vi "Register for gRPC Server Events.vi"(8 "error in (no error)":errorcluster, 11 "CIFPlugin in":refnum<class "CAN_Reader_CANsub_Plugin.lvclass">) -> (0 "error out":errorcluster, 2 "Event Registration Refnum":refnum<event-registration>, 3 "CIFPlugin out":refnum<class "CAN_Reader_CANsub_Plugin.lvclass">)   [LabVIEW 2021, in "CAN_Reader_CANsub_Plugin.lvclass"]
uses:
  CAN_Reader_CANsub_Plugin.lvclass
  CAN_Reader_CANsub_Plugin.lvclass/CAN_Reader_CANsub_Plugin.ctl
  <vilib>/CIF Foundation/CIF Core/CIFCore/Class/CIFCorePlugin.lvclass
  Grpc/CanReaderCansub_server/RPC Service/CanReaderCansub/CanReaderCansub.lvclass
  C:/Program Files/National Instruments/LabVIEW 2021/vi.lib/CIF Foundation/CIF Core/CIFCore/Class/CIFCorePlugin.lvclass
  D:/dev/Plugins/CAN_Reader_CANsub/Class/CAN_Reader_CANsub_Plugin.lvclass
  <vilib>/CIF Foundation/CIF U8 Array Monitor gRPC/U8_Array_Monitor_gRPC/CIFU8ArrayMonitorUtilities/CIFU8ArrayMonitorUtilities.lvlib
  C:/Program Files/National Instruments/LabVIEW 2021/vi.lib/gRPC/LabVIEW gRPC Servicer/ServiceBase/ServiceBase.lvclass
  D:/dev/Plugins/CAN_Reader_CANsub/Grpc/CanReaderCansub_server/RPC Service/CanReaderCansub/CanReaderCansub.lvclass
  <vilib>/gRPC/LabVIEW gRPC Library/Shared/grpcId.ctl
  <vilib>/gRPC/LabVIEW gRPC Library/grpc-lvsupport-release.lvlib
  <vilib>/gRPC/LabVIEW gRPC Library/Server API/typeDefs/gRPCId Cluster.ctl
  <vilib>/CIF Foundation/CIF U8 Array Monitor gRPC/U8_Array_Monitor_gRPC/CIFU8ArrayMonitor_server/RPC Service/U8ArrayMonitor/typeDefs/Server gRPC UEs.ctl
  <vilib>/CIF Foundation/CIF U8 Array Monitor gRPC/U8_Array_Monitor_gRPC/CIFU8ArrayMonitor_server/RPC Service/U8ArrayMonitor/U8ArrayMonitor.lvclass
  Grpc/CanReaderCansub_server/RPC Service/CanReaderCansub/typeDefs/Server gRPC UEs.ctl
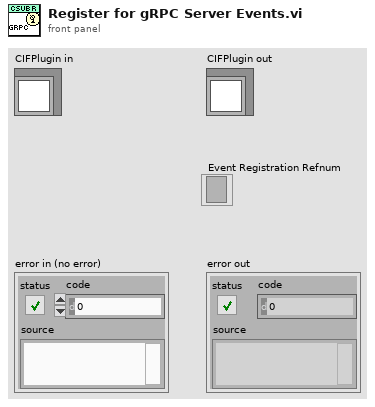
[diagram p1: front panel]
types:
  T1 = typedef "CIFU8ArrayMonitor_server.lvlib/U8ArrayMonitor.lvclass/Server gRPC UEs.ctl" = cluster{"U8ArrayMonitor SetEnableU8Array gRPC UE":refnum<user-event>, "U8ArrayMonitor GetU8Array gRPC UE":refnum<user-event>}
  T2 = typedef "CanReaderCansub_server.lvlib/CanReaderCansub.lvclass/Server gRPC UEs.ctl" = cluster{"CanReaderCansub GetDevices gRPC UE":refnum<user-event>, "CanReaderCansub GetStatistics gRPC UE":refnum<user-event>, "CanReaderCansub SetInterfaceBlink gRPC UE":refnum<user-event>, "CanReaderCansub GetCANStatus gRPC UE":refnum<user-event>}
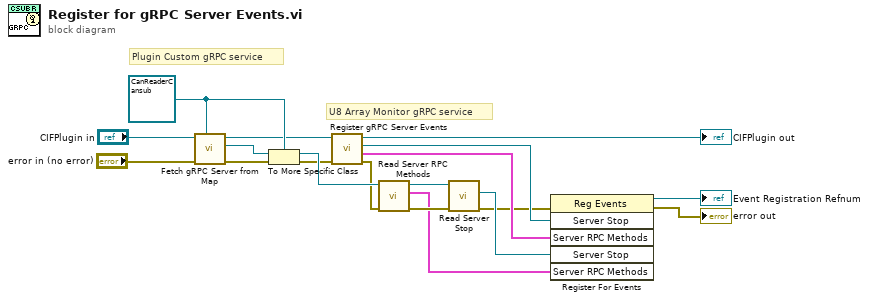
[diagram p0: block diagram]
diagram:
  w11 = refnum<class "CanReaderCansub.lvclass"> refnum ("CanReaderNixnet")
  # "U8 Array Monitor gRPC service"
  # "Plugin Custom gRPC service"
  n1 = call <vilib>:"Fetch gRPC Server from Map.vi"("gRPC Server Class type"=w11, "error in (no error)"="error in (no error)", "CIFCorePlugin in"="CIFPlugin in") -> ("error out"=w15:errorcluster, "gRPC Server Class out"=w14:refnum<class "ServiceBase.lvclass">, "CIFCorePlugin out"=w8:refnum<class "CAN_Reader_CANsub_Plugin.lvclass">)  [unwired: 6 in]
  n2 = To More Specific Class(target class=w11, reference=w14, error in=w15) -> (specific class reference=w16:refnum<class "CanReaderCansub.lvclass">, error out=w7:errorcluster)
  n3 = call <vilib>:"Register gRPC Server Events.vi"("error in"=w7, "CIFPlugin in"=w8) -> ("error out"=w5:errorcluster, "Server RPC Methods"=w3:T1, "Server Stop"=w4:refnum<user-event>, "CIFPlugin out"=→"CIFPlugin out":refnum<class "CAN_Reader_CANsub_Plugin.lvclass">)  [unwired: 6 in]
  n4 = call "Read Server RPC Methods.vi"("error in (no error)"=w5, "gRPC service in"=w16) -> ("error out"=w17:errorcluster, "Server RPC Methods"=w10:T2, "gRPC service out"=w18:refnum<class "CanReaderCansub.lvclass">)  [unwired: 7 in]
  n5 = call-dynamic "Read Server Stop.vi"("error in"=w17, "gRPC service in"=w18) -> ("error out"=w2:errorcluster, "Server Stop"=w9:refnum<user-event>)  [unwired: 7 in, 1 out]
  n6 = register-events(error in=w2, w4, w3, w9, w10) -> (reference out=→"Event Registration Refnum":refnum<event-registration>, error out=→"error out":errorcluster)  [unwired: 1 in]
